vi "VIH Project Tree - Sort Items.vi"(8 "error in":errorcluster, 9 "Recursively (T)":bool=TRUE, 10 "Parent Tag":string, 11 "Project Tree":T1) -> (0 "error out":errorcluster, 2 "dup Parent Tag":string, 3 "dup Project Tree":T1)   [LabVIEW 2014]
doc: "::: VI Helpeks :::\nCopyright (c) 2000-2026 Konstantin Shifershteyn. All rights reserved."
uses:
  VIH Project Tree Typedef - Tree Refnum.ctl
panel:
  # "VI Helpeks\nCopyright (c) 2012-2026 Konstantin Shifershteyn"
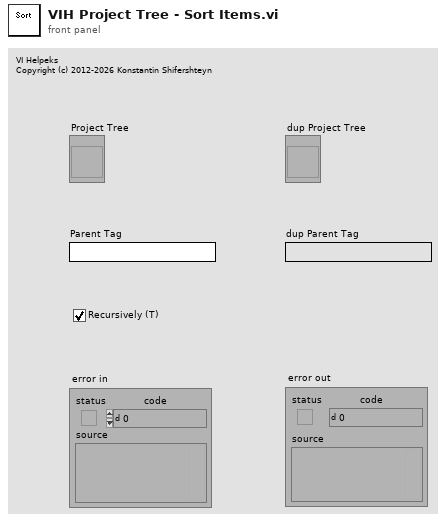
[diagram p1: front panel]
types:
  T1 = typedef "VIH Project Tree Typedef - Tree Refnum.ctl" = refnum<vi>
  T2 = typedef "VIH Project Tree Typedef - Tree Item Type.ctl" = enum32{"<Invalid>", "Project", "Proj Files", "Proj Rules", "File Group", "Rule Group", "Any File", "LV Func", ".mnu", ".mnu (dyn)", ".vi", ".vi (dyn)", ".vit", ".vit (dyn)", ".ctl", ".ctl (dyn)", ".ctt", ".ctt (dyn)", "polyVI", "polyVI (dyn)", "expVI", "expVI (dyn)", "HTML", "PolyVI Inst"}
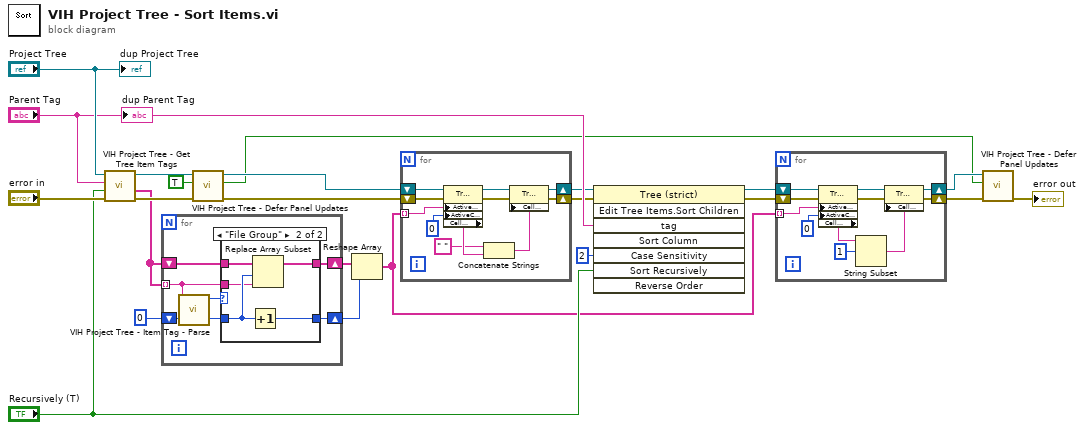
[diagram p0: block diagram]
diagram:
  n1 = call "VIH Project Tree - Get Tree Item Tags.vi"("error in"="error in", "Recursively (T)"="Recursively (T)", "Parent Item Tag"="Parent Tag", "Project Tree"="Project Tree") -> ("error out"=w19:errorcluster, "Child Item Tags"=w15:string[], "dup Project Tree"=w20:T1)  [unwired: 4 in, 1 out]
  n2 = for {
    tunnel: w15 -> [w24] mode=indexing
    shift-right: [w28] -> w13
    shift-left: w15 -> [w27]
    shift-right: [w26] -> w12
    shift-left: 0 -> [w25]
    n3 = call "VIH Project Tree - Item Tag - Parse.vi"("Tree Item Tag"=w24) -> ("Item Type"=w29:T2)  [unwired: 8 in, 2 out]
    n4 = case shown="\"File Group\"" w29 {
      tunnel: [w31 w33] -> w28
      tunnel: w27 -> [w31 w36]
      tunnel: [w30 w34] -> w26
      tunnel: w25 -> [w30 w35]
      tunnel: w24 -> [_ w32]
      frame Default {
      }
      frame "File Group" {
        n5 = Increment(x=w35) -> (x+1=w34:i32)
        n6 = Replace Array Subset(array=w36, new element=w32, index=w35) -> (w33:string[])
      }
    }
  }
  n7 = call "VIH Project Tree - Defer Panel Updates.vi"("error in"=w19, "Defer Panel Updates (F)"=TRUE, "Project Tree"=w20) -> ("error out"=w11:errorcluster, "Previous Defer status"=w1:bool, "dup Project Tree"=w10:T1)  [unwired: 6 in]
  n8 = Reshape Array(w13, w12) -> (w5:string[])
  n9 = for {
    shift-right: [w38] -> w9
    shift-left: w11 -> [w47]
    shift-right: [w37] -> w8
    shift-left: w10 -> [w46]
    tunnel: w5 -> [w45] mode=indexing
    n10 = property class="Tree (strict)"(reference=w46, error in=w47, "Active Item Tag"=w45, "ActiveColNum"=0 ("Active Cell:Active Column Number")) -> (reference out=w43:T1, error out=w42:errorcluster, "Cell String"=w41:string)
    n11 = Concatenate Strings(" " ("string"), w41) -> (w39:string)
    n12 = property class="Tree (strict)"(reference=w43, error in=w42, "Cell String"=w39) -> (reference out=w37:T1, error out=w38:errorcluster)
  }
  n13 = invoke on="Invoke Node" class="Tree (strict)" method="Edit Tree Items.Sort Children"(reference=w8, error in=w9, "tag"="Parent Tag", "Case Sensitivity"=2, "Sort Recursively"="Recursively (T)") -> (reference out=w7:T1, error out=w6:errorcluster)  [unwired: 3 in, 6 out]
  n14 = for {
    shift-right: [w52] -> w4
    shift-left: w6 -> [w58]
    shift-right: [w51] -> w3
    shift-left: w7 -> [w57]
    tunnel: w5 -> [w56] mode=indexing
    n15 = property class="Tree (strict)"(reference=w57, error in=w58, "Active Item Tag"=w56, "ActiveColNum"=0 ("Active Cell:Active Column Number")) -> (reference out=w54:T1, error out=w53:errorcluster, "Cell String"=w50:string)
    n16 = String Subset(string=w50, offset (0)=1) -> (substring=w49:string)  [unwired: 1 in]
    n17 = property class="Tree (strict)"(reference=w54, error in=w53, "Cell String"=w49) -> (reference out=w51:T1, error out=w52:errorcluster)
  }
  n18 = call "VIH Project Tree - Defer Panel Updates.vi"("error in"=w4, "Defer Panel Updates (F)"=w1, "Project Tree"=w3) -> ("error out"=→"error out":errorcluster)  [unwired: 6 in, 2 out]
  "dup Project Tree" <- "Project Tree"
  "dup Parent Tag" <- "Parent Tag"
